vi "Get Class Inheritance from Class Path.vi"(8 "error in (no error)":errorcluster, 11 "lvclass file Path":path) -> (0 "error out":errorcluster, 3 "Class Inheritance [ ]":path[](array[path]))   [LabVIEW 2013, in "VITesterUtilities.lvlib"]
uses:
  Libraries/VITesterUtilities.lvlib
  <vilib>/Utility/lvfile.llb/LVFileType.ctl
  <userlib>/_OpenG.lib/file/file.llb/File Exists - Scalar__ogtk.vi
  <userlib>/_OpenG.lib/file/file.llb/Valid Path - Traditional__ogtk.vi
  <userlib>/_OpenG.lib/array/array.llb/Conditional Auto-Indexing Tunnel (Path)__ogtk.vi
  <userlib>/_OpenG.lib/file/file.llb/Append Path to Root if Relative - Scalar__ogtk.vi
  <vilib>/Utility/lvfile.llb/NI_FileType.lvlib
panel:
  # "Copyright © 2008 James Kring, Inc. All rights reserved.\n\nAuthor: Philippe Guerit [philippe.guerit@jameskring.com]\n             [alternate email: PJM_LabVIEW@yahoo.com]\n\nThis library is provided \"AS IS\" ,WITHOUT WARRANTIES OR \nCONDITIONS OF ANY KIND, either express or implied.\n\nJames Kring, Inc. -- http://www.jameskring.com"
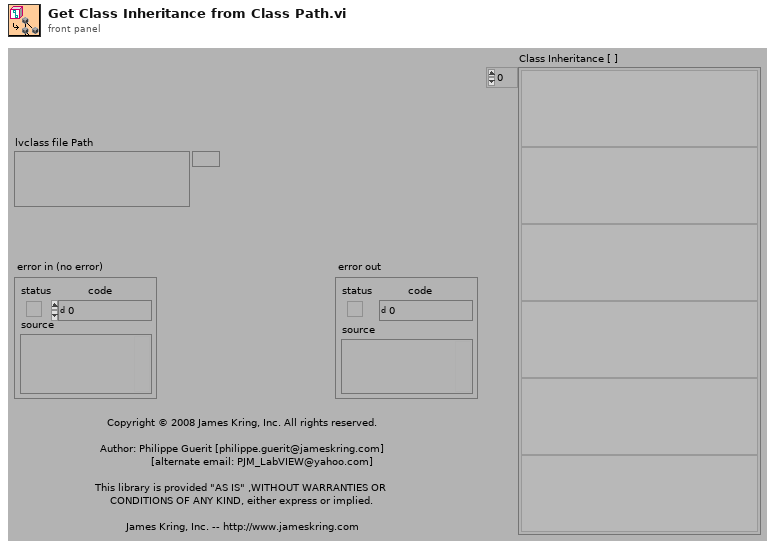
[diagram p1: front panel]
types:
  T1 = typedef "NI_FileType.lvlib/LVFileType.ctl" = enum32{"Invalid file", "Unknown type", "Instrument", "Control", "Polymorphic VI", "Project", "Library", "LVClass", "XControl", "XNode", "Shared library", ".NET assembly", "ActiveX interface", "CIN", "Run-time menu", "Palette menu", "Help file", "LLB", "XNode Edit Dependency", "Class Private Data Control", "Statechart", "MathScript .m file", "Ladder Diagram", "LVLibp", "XNode Build Dependency"}
  T2 = typedef "NI_FileType.lvlib/LVFileType.ctl" = enum32{"Invalid file", "Unknown type", "Instrument", "Control", "Polymorphic VI", "Project", "Library", "LVClass", "XControl", "XNode", "Shared library", ".NET assembly", "ActiveX interface", "CIN", "Run-time menu", "Palette menu", "Help file", "LLB", "XNode Edit Dependency", "Class Private Data Control", "Statechart", "MathScript .m file", "Ladder Diagram", "LVLibp"}
  T3 = cluster{"path":path, "delimited name":string, "type":T2, "iState":u32, "iStyle":u16, "wStyle":u16, "buttons":u16, "viflags":u32, "viflags2":u32, "links":u32[]}[]
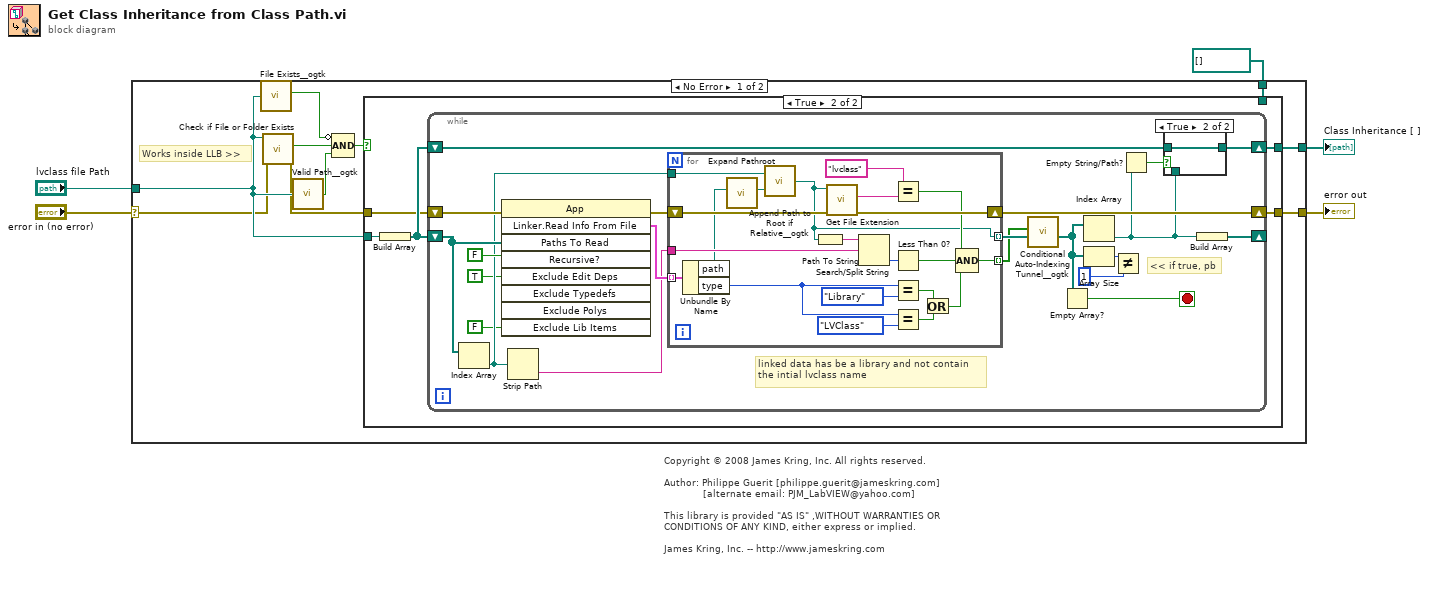
[diagram p0: block diagram]
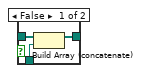
[diagram p3: hidden frame]
diagram:
  # "Copyright © 2008 James Kring, Inc. All rights reserved.\n\nAuthor: Philippe Guerit [philippe.guerit@jameskring.com]\n             [alternate email: PJM_LabVIEW@yahoo.com]\n\nThis library is provided \"AS IS\" ,WITHOUT WARRANTIES OR \nCONDITIONS OF ANY KIND, either express or implied.\n\nJames Kring, Inc. -- http://www.jameskring.com"
  n1 = case shown="No Error" "error in (no error)" {
    selector: "error in (no error)" -> [w7 w70]
    tunnel: [w15 w69] -> w5
    tunnel: "lvclass file Path" -> [w8 _]
    tunnel: [w14 w70] -> w2
    tunnel: path[] [] -> [w10 w69]
    frame No Error {
      # "Works inside LLB >>"
      n2 = call-poly <userlib>:"File Exists__ogtk.vi"("file path"=w8) -> ("is directory"=w13:bool)  [unwired: 6 in, 1 out]
      n3 = call <vilib>:"Check if File or Folder Exists.vi"("error in (no error)"=w7, "path"=w8) -> ("error out"=w6:errorcluster, "file or folder exists?"=w9:bool)  [unwired: 7 in, 1 out]
      n4 = call-poly <userlib>:"Valid Path__ogtk.vi"("path"=w8) -> ("valid"=w12:bool)
      n5 = Compound Arithmetic op=AND(invert w13, w9, w12) -> (w11:bool)
      n6 = case shown="True" w11 {
        tunnel: [w16 w21] -> w15
        tunnel: w6 -> [w17 w20]
        tunnel: [w17 w19] -> w14
        tunnel: w8 -> [_ w18]
        tunnel: w10 -> [w16 _]
        frame False {
        }
        frame True {
          n7 = Build Array(w18) -> (w22:path[])
          n8 = while {
            shift-right: [w31] -> _
            shift-left: w22 -> [w32]
            shift-right: [w33] -> w21
            shift-left: w22 -> [w34]
            shift-right: [w28] -> w19
            shift-left: w20 -> [w30]
            stop <- w35 stop-if-true
            # "<< if true, pb"
            # "linked data has be a library and not contain\nthe intial lvclass name"
            n9 = Index Array(array=w32) -> (element=w25:path)  [unwired: 1 in]
            n10 = invoke class="App" method="Linker.Read Info From File"(error in=w30, "Paths To Read"=w32, "Recursive?"=FALSE, "Exclude Edit Deps"=TRUE ("Exclude Edit Time Dependencies"), "Exclude Lib Items"=FALSE ("Exclude Unused Library Items")) -> (error out=w29:errorcluster, "Linker.Read Info From File"=w42:T3)  [unwired: 4 in, 7 out]
            n11 = Strip Path(path=w25) -> (name=w41:string)  [unwired: 1 out]
            n12 = for {
              tunnel: w42 -> [w68] mode=indexing
              tunnel: w41 -> [w65]
              tunnel: [w53] -> w40 mode=indexing
              tunnel: [w62] -> w39 mode=indexing
              shift-right: [w60] -> w28
              shift-left: w29 -> [w61]
              tunnel: w25 -> [w55]
              n13 = Unbundle By Name(w68) -> ("path"=w54:path, "type"=w51:T2)
              n14 = call "Expand Pathroot.vi"("Path"=w54) -> ("Path out"=w56:path)  [unwired: 10 in]
              n15 = call-poly <userlib>:"Append Path to Root if Relative__ogtk.vi"("Absolute or Relative Path"=w56, "Root Path"=w55) -> ("Absolute or Appended Path"=w53:path)
              n16 = Path To String(path=w53) -> (string=w66:string)
              n17 = call <vilib>:"Get File Extension.vi"("error in (no error)"=w61, "file"=w53) -> ("error out"=w60:errorcluster, "lowercase file extension"=w57:string)  [unwired: 8 out]
              n18 = Search/Split String(string=w66, search string/char (-)=w65) -> (offset of match=w64:i32)  [unwired: 3 out]
              n19 = Equal?(x="lvclass", y=w57) -> (x = y?=w58:bool)
              n20 = Less Than 0?(x=w64) -> (x < 0?=w63:bool)
              n21 = Equal?(x=w51, y=LVFileType."Library") -> (x = y?=w49:bool)
              n22 = Equal?(x=w51, y=LVFileType."LVClass") -> (x = y?=w50:bool)
              n23 = Or(x=w49, y=w50) -> (x .or. y?=w48:bool)
              n24 = Compound Arithmetic op=AND(w58, w63, w48) -> (w62:bool)
            }
            n25 = call-poly <userlib>:"Conditional Auto-Indexing Tunnel__ogtk.vi"("Array in"=w40, "Elements to keep"=w39) -> ("Filtered Array out"=w36:path[])  [unwired: 5 out]
            n26 = Empty Array?(array=w36) -> (empty?=w35:bool)
            n27 = Index Array(array=w36) -> (element=w27:path)  [unwired: 1 in]
            n28 = Array Size(array=w36) -> (size(s)=w38:i32)
            n29 = Not Equal?(x=w38, y=1) -> ()  [unwired: 1 out]
            n30 = Empty String/Path?(string/path=w27) -> (empty?=w26:bool)
            n31 = case shown="True" w26 {
              tunnel: w34 -> [w46 w47]
              tunnel: [w45 w47] -> w33
              tunnel: w27 -> [w44 _]
              frame False {
                n32 = Build Array (concatenate)(w46, w44) -> (w45:path[])
              }
              frame True {
              }
            }
            n33 = Build Array(w27) -> (w31:path[])
          }
        }
      }
    }
    frame Error {
    }
  }
  "Class Inheritance [ ]" <- w5
  "error out" <- w2
